vi "Stop Condition - Saturation 4 (SubVI) (1).vi"(6 "Enum":T1(ring), 8 "error in (no error)":errorcluster, 9 "Time":dbl, 11 "Cluster in":T2 {"M Event" items=["Stop", "Running", "PID", "Up Limit", "Down Limit", "Load Limit"]; "Test Type" items=["Please Select", "Triaxial Shear", "Triaxial UU", "Shearbox", "Permeability", "Consolidation (Stepped Loading)/Swelling", "Saturation (Incremental)", "User Defined", "UCT", "Isotropic Consolidation", "Swelling Pressure", "B-Check", "Saturation (Step Increment)", "Saturation (Ramp)"]; "Data"."Test Type" items=["Please Select", "Triaxial Shear", "Triaxial UU", "Shearbox", "Permeability", "Consolidation (Stepped Loading)/Swelling", "Saturation (Incremental)", "User Defined", "UCT", "Isotropic Consolidation", "Swelling Pressure", "B-Check", "Saturation (Step Increment)", "Saturation (Ramp)"]}) -> (0 "error out":errorcluster, 3 "Cluster out":T2 {"M Event" items=["Stop", "Running", "PID", "Up Limit", "Down Limit", "Load Limit"]; "Test Type" items=["Please Select", "Triaxial Shear", "Triaxial UU", "Shearbox", "Permeability", "Consolidation (Stepped Loading)/Swelling", "Saturation (Incremental)", "User Defined", "UCT", "Isotropic Consolidation", "Swelling Pressure", "B-Check", "Saturation (Step Increment)", "Saturation (Ramp)"]; "Data"."Test Type" items=["Please Select", "Triaxial Shear", "Triaxial UU", "Shearbox", "Permeability", "Consolidation (Stepped Loading)/Swelling", "Saturation (Incremental)", "User Defined", "UCT", "Isotropic Consolidation", "Swelling Pressure", "B-Check", "Saturation (Step Increment)", "Saturation (Ramp)"]}, 4 "Delay":string, 7 "Log?":bool)   [LabVIEW 2019]
uses:
  Controls/RunTest - Data Structure.ctl
  Controls/Test Panel - Data Structure.ctl
  Controls/Station - Test Type.ctl
  <vilib>/Utility/miscctls.llb/LVRowAndColumnTypeDef.ctl
  Controls/RunTest - Calculate Data.ctl
  <vilib>/httpClient/ClientHandle.ctl
  Controls/RunTest - Start Condition.ctl
  Controls/RunTest - Stop Condition.ctl
  Controls/UDP - Event.ctl
  Controls/RunTest - State.ctl
  Controls/eFGV States.ctl
  <vilib>/httpClient/LabVIEWHTTPClient.lvlib
types:
  T1 = enum16{"Saturation", "B-Check", "Sat Step", "Sat Ramp"}
  T2 = typedef "RunTest - Data Structure.ctl" = cluster{"Test Plan":string[], "PlanRow":i32, "Device Name":string[], "Timeout":i32, "Start?":bool, "Pause?":bool, "IP Address":string[], "LogRow":i32, "Logtype":u16, "Log Elapse":sgl, "Data":T3, "Stop log?":bool, "tdms":refnum<k34>, "Sensor Data":sgl[], "Start time":timestamp, "Prev Log Elapse":u32, "Plot":u16, "X-Axis":u16[], "Y-Axis":u16[], "XY":cluster{"X":dbl, "Y":dbl}[][], "End Stage?":bool, "1run":bool, "Condition":u16[], "Start Con":bool, "Log Con":bool, "Stop Con":bool, "Start Elapse":dbl, "Start Load":dbl, "Motor":i32, "StartRow":i32, "number log":i32, "Dir":bool, "Start time test":timestamp, "Auto":bool, "Check return?":bool, "Inv":cluster{"M":i32[], "Bool":bool[]}, "tdms temp":refnum<k34>, "Zero?":bool, "Plot Timer":dbl, "1st Run":bool, "TDMS Path":path, "MaxLoad":dbl, "Log Timer":sgl[], "Test Type":T4, "Log Sensor":string[], "Save?":bool, "1st Log":bool, "Y-Axis 2":u16[], "On Y-Axis 2":bool, "Decimal":u8[], "Init":cluster{"PWP TS":sgl, "Load TS":sgl, "Volume TS":sgl, "Disp TS":sgl, "CP":sgl, "Vol In":sgl, "Vol Out":sgl, "Load UCT":sgl, "Disp UCT":sgl, "PWP Sat":sgl, "CP Sat":sgl, "Volume IsoCons":sgl, "PWP IsoCons":sgl, "PWP TUU":sgl, "Load TUU":sgl, "Volume TUU":sgl, "Disp TUU":sgl, "Load Cons":sgl, "Disp Cons":sgl, "Volume Sat":sgl, "Vertical Load SB":sgl, "Vertical Disp SB":sgl, "H Disp SB":sgl, "H Load SB":sgl, "PWP BC":sgl, "CP BC":sgl, "PWP Sat Step":sgl, "CP Sat Step":sgl, "Volume Sat Step":sgl, "PWP Sat Ramp":sgl, "CP Sat Ramp":sgl, "Volume Sat Ramp":sgl}, "Calc":T6, "Device Index":i32[], "Channel Index":i32[], "http ref":T7, "fileid":string, "Step Cons":cluster{"V Stress":sgl, "H Settlement":sgl}, "RunTest":bool, "Graph Last":i32, "Init?":bool, "Datalog":bool[], "Start":T8, "Stop":T9, "Running?":bool, "StartTime":dbl, "Log Prev Time":dbl, "KeyName":string[], "Test RunTime":dbl, "Log Prev Axial":dbl, "M Event":T10[], "Last Log":bool, "popup":bool, "PreStart UU":bool, "PreStart Sat":bool, "PreStart BC":bool, "PreStart Sat Step":bool, "PreStart Sat Ramp":bool, "Prev Sat IP":string}
  T3 = typedef "Test Panel - Data Structure.ctl" = cluster{"Station":string, "Sample ID":string, "Job No":string, "Job Description":string, "Filename":string, "Test Type":T4, "Speciment No":string, "Depth":string, "Height":string, "Diameter/Length":string, "Weight":string, "Test Parameter":string, "Station[]":string[], "Edit Pos":T5, "Edit Pos Prev":T5, "Area":string, "Path":string, "sample_id":string}
  T4 = typedef "Station - Test Type.ctl" = u16
  T5 = typedef "LVRowAndColumnTypeDef.ctl" = cluster{"Row":i32, "Column":i32}
  T6 = typedef "RunTest - Calculate Data.ctl" = cluster{"TS":cluster{"Change PWP":sgl, "Change Vol":sgl, "Axial Load":sgl, "CiL":sgl, "Deviator":sgl, "Axial Strain":sgl, "MaxDeviator":sgl, "SS":sgl, "CAS":sgl}, "TUU":cluster{"Change PWP":sgl, "Axial Load":sgl, "CiL":sgl, "Deviator":sgl, "Axial Strain":sgl, "MaxDeviator":sgl}, "Sat":cluster{"B Value":sgl, "PWP Diss":sgl, "CPP":sgl, "CV":sgl}, "Per":cluster{"Change Vol In":sgl, "Change Vol Out":sgl, "Mean Vol":sgl, "Gradient Pressure":sgl, "Outlet Flow":sgl, "Inlet Flow":sgl, "I X1":sgl, "I X2":sgl, "I Y1":sgl, "I Y2":sgl, "O X1":sgl, "O X2":sgl, "O Y1":sgl, "O Y2":sgl}, "Step Cons":cluster{"V Stress":sgl, "H Settlement":sgl, "Total H Settle":sgl, "Prev Total H":sgl}, "UCT":cluster{"ALC":sgl, "H Change":sgl, "Deviator":sgl, "Axial Strain":sgl, "V Stress":sgl, "MaxDeviator":sgl}, "ISO Cons":cluster{"CPP":sgl, "PWP Diss":sgl, "CV":sgl, "VS":sgl}, "SB":cluster{"Speci LenC":sgl, "Shear Strain":sgl, "H LC":sgl, "Normal Stress":sgl, "Shear Stress":sgl, "MaxShear":sgl}, "BC":cluster{"B Value":sgl, "PWP Diss":sgl, "CPP":sgl, "CV":sgl}, "Sat Step":cluster{"B Value":sgl, "PWP Diss":sgl, "CPP":sgl, "CV":sgl}, "Sat Ramp":cluster{"B Value":sgl, "PWP Diss":sgl, "CPP":sgl, "CV":sgl}, "Prev Log":string[]}
  T7 = typedef "LabVIEWHTTPClient.lvlib/ClientHandle.ctl" = refnum<k1>
  T8 = typedef "RunTest - Start Condition.ctl" = cluster{"Cons":cluster{"VS":dbl, "Delay":bool, "No Delay":dbl}, "Sat":cluster{"CP":dbl, "BP":dbl, "StartBP":bool, "Target CP":bool, "Target BP":bool}, "Iso":cluster{"Select":dbl, "BP":dbl, "IC2":dbl, "IC3":dbl, "IC4":dbl, ". IC6":bool, "IC6":dbl, "IC6-2":dbl, "Time Cond":dbl, "Last PWP":dbl, "Target CP":bool, "Target BP":bool, "NewCP":dbl, "NewBP":dbl, "Noti CP":bool, "Noti BP":bool, "Noti PWP":bool, "PrevSatBP":dbl}, "TS":cluster{"SS":dbl, "Engage":bool, "ES":dbl, "LC":dbl, "PreStart":bool, "Trig SS":bool, "Drain":dbl, "Select":u16, "Max SS .":bool, "MaxSS":dbl}, "TUU":cluster{"SS":dbl, "Engage":bool, "ES":dbl, "LC":dbl, "PreStart":bool, "Trig SS":bool, "CP":dbl, "Delay Value":dbl, "Delay":bool, "CP PID":bool}, "UCT":cluster{"SS":dbl, "Engage":bool, "ES":dbl, "LC":dbl, "PreStart":bool, "Trig SS":bool}, "Enable?":bool, "SB":cluster{"SS":dbl, "Engage":bool, "ES":dbl, "LC":dbl, "PreStart":bool, "Trig SS":bool, "VS":dbl, "Delay Value":dbl, "Delay":bool, "VS PID":bool}, "Perm":cluster{"DP":dbl}, "BC":cluster{"CP":dbl, "Target CP":bool, "Target BP":bool, "CP Inc":dbl, "CP .Init":bool, "CP Init":dbl, "1st BC":bool}, "Sat (Step)":cluster{"Select":dbl, "CP":dbl, "BP":dbl, "EP":dbl, "StartCP":bool, "Target CP":bool, "Target BP":bool}, "Sat (Ramp)":cluster{"Select":dbl, "CP":dbl, "BP":dbl, "EP":dbl, "StartCP":bool, "Target CP":bool, "Target BP":bool, "Time Rate":u32}}
  T9 = typedef "RunTest - Stop Condition.ctl" = cluster{"Cons":cluster{"Select":i32, "Disp":dbl, "Time":dbl, "Time2":dbl, "Disp 2":dbl, "Time Cond":dbl, "Last Disp":dbl, "Swell":bool, "T50,90,100":cluster{"t50_x_min":dbl, "t50_y_value":dbl, "t90_x_min":dbl, "t90_y_value":dbl, "t100_x_min":dbl, "t100_y_value":dbl, "target_column":string, "test_type":string, "error":string}}, "Sat":cluster{"Select":i32, "PP":dbl, "Time":dbl, "VC":dbl, "Time2":dbl, "Time Cond":dbl, "Last PP":dbl, ".B":bool, "B":dbl, "Last Vc":dbl, "Time Cond 2":dbl, "Time3":dbl, "Time Cond 3":dbl, "B Achieve":bool, "PP Achieve":bool, "VC Achieve":bool, "Max Achieve":bool, "CP Check":dbl, "Skip Next":bool, "B Achieve Stage":u32, ".CP Check":bool}, "Iso":cluster{"PP":dbl, "Time":dbl, "VC":dbl, "Time2":dbl, "Time Cond":dbl, "Last Vc":dbl, ".PP":bool, "Time Cond 2":dbl, "Select":i32, "BS":cluster{"t50_x_min":dbl, "t50_y_value":dbl, "t90_x_min":dbl, "t90_y_value":dbl, "t100_x_min":dbl, "t100_y_value":dbl, "target_column":string, "test_type":string, "error":string}, "Final VC":dbl, "ASTM":cluster{"t50_x_min":dbl, "t50_y_value":dbl, "t90_x_min":dbl, "t90_y_value":dbl, "t100_x_min":dbl, "t100_y_value":dbl, "target_column":string, "test_type":string, "error":string}, "ASTM Log":cluster{"t50_x_min":dbl, "t50_y_value":dbl, "t90_x_min":dbl, "t90_y_value":dbl, "t100_x_min":dbl, "t100_y_value":dbl, "target_column":string, "test_type":string, "error":string}, "PP Achieve":bool, "VC Achieve":bool}, "TS":cluster{"Axial":dbl, ".MaxDev":bool, "MaxDev Value":dbl, "Return":bool, "Reset":bool, "Prev Time":dbl, "PostStop Run":bool, "CP Stop":bool, "BP Stop":bool, "PostStop Trig":bool, "Reset Value":dbl, "BPTrig":bool, "CPTrig":bool, "VLCTrig":bool, "CAxial":dbl, "Select":i32}, "TUU":cluster{"Axial":dbl, ".MaxDev":bool, "MaxDev Value":dbl, "Return":bool, "Reset":bool, "Prev Time":dbl, "PostStop Run":bool, "CP Stop":bool, "BP Stop":bool, "PostStop Trig":bool, "Reset Value":dbl, "BPTrig":bool, "CPTrig":bool, "VLCTrig":bool}, "UCT":cluster{"Axial":dbl, ".MaxDev":bool, "MaxDev Value":dbl, "Return":bool, "Reset":bool, "Prev Time":dbl, "PostStop Run":bool, "CP Stop":bool, "BP Stop":bool, "PostStop Trig":bool}, "Enable?":bool, "SB":cluster{"Shear":dbl, ".MaxShear":bool, "MaxShear Value":dbl, "Return":bool, "Reset":bool, "Prev Time":dbl, "PostStop Run":bool, "CP Stop":bool, "BP Stop":bool, "PostStop Trig":bool, "Reset Value":dbl, "BPTrig":bool, "CPTrig":bool, "VLCTrig":bool}, "Perm":cluster{"Max Time":bool, "Reset":bool, "PostStop Run":bool, "Ratio":bool, "Reset Value":dbl, "Time":dbl, "RatioTime":dbl, "RatioMore":dbl, "RatioLess":dbl, "Time Cond":dbl, "Time Cond 2":dbl, "Prev IF":dbl, "Prev OF":dbl, "PostStop Trig":bool, "BP Trig":bool, "DP Stop":bool, "BP Stop":bool, "CP Stop":bool, "CP Trig":bool}, "SP":cluster{".Max Time":bool, ".Time":bool, "Time":dbl, "MaxTime":dbl, "Time Cond":dbl, "Max Time Cond":dbl, "Stress":dbl}, "BC":cluster{"Select":i32, "PP":dbl, "Time":dbl, "Time Cond":dbl, "Last PP":dbl, ".B":bool, "B":dbl, "Time 2":dbl, "Time Cond 2":dbl, "B Achieve":bool, "PP Achieve":bool, "Max Achieve":bool, "CP Check":dbl, "Skip Next":bool, "B Achieve Stage":u32, ".CP Check":bool}, "Sat (Step)":cluster{"Select":i32, "PP":dbl, "Time":dbl, "VC":dbl, "Time2":dbl, "Time Cond":dbl, "Last PP":dbl, ".B":bool, "B":dbl, "Last Vc":dbl, "Time Cond 2":dbl, "Time3":dbl, "Time Cond 3":dbl, "B Achieve":bool, "PP Achieve":bool, "VC Achieve":bool, "Max Achieve":bool, "CP Check":dbl, "Skip Next":bool, "B Achieve Stage":u32}, "Sat (Ramp)":cluster{"Select":i32, "PP":dbl, "Time":dbl, "VC":dbl, "Time2":dbl, "Time Cond":dbl, "Last PP":dbl, ".B":bool, "B":dbl, "Last Vc":dbl, "Time Cond 2":dbl, "Time3":dbl, "Time Cond 3":dbl, "B Achieve":bool, "PP Achieve":bool, "VC Achieve":bool, "Max Achieve":bool, "CP Check":dbl, "Skip Next":bool, "B Achieve Stage":u32}}
  T10 = typedef "UDP - Event.ctl" = u16
  T11 = typedef "RunTest - State.ctl" = enum16{"Load Testfile", "Notifier", "Init", "Idle", "Load", "Read DB", "Run", "Pause", "Stop", "Check Start", "Check Stop", "Check Post Stop", "Check Log", "EndStage", "Data View", "Data View PWP", "Display", "Graph", "Graph PWP", "Close", "Stop PID", "Check Limit", "Auto", "Up", "Log", "Zero", "Machine Control", "Save Report"}
  T12 = typedef "eFGV States.ctl" = enum16{"Init", "Read", "Write", "Exit"}
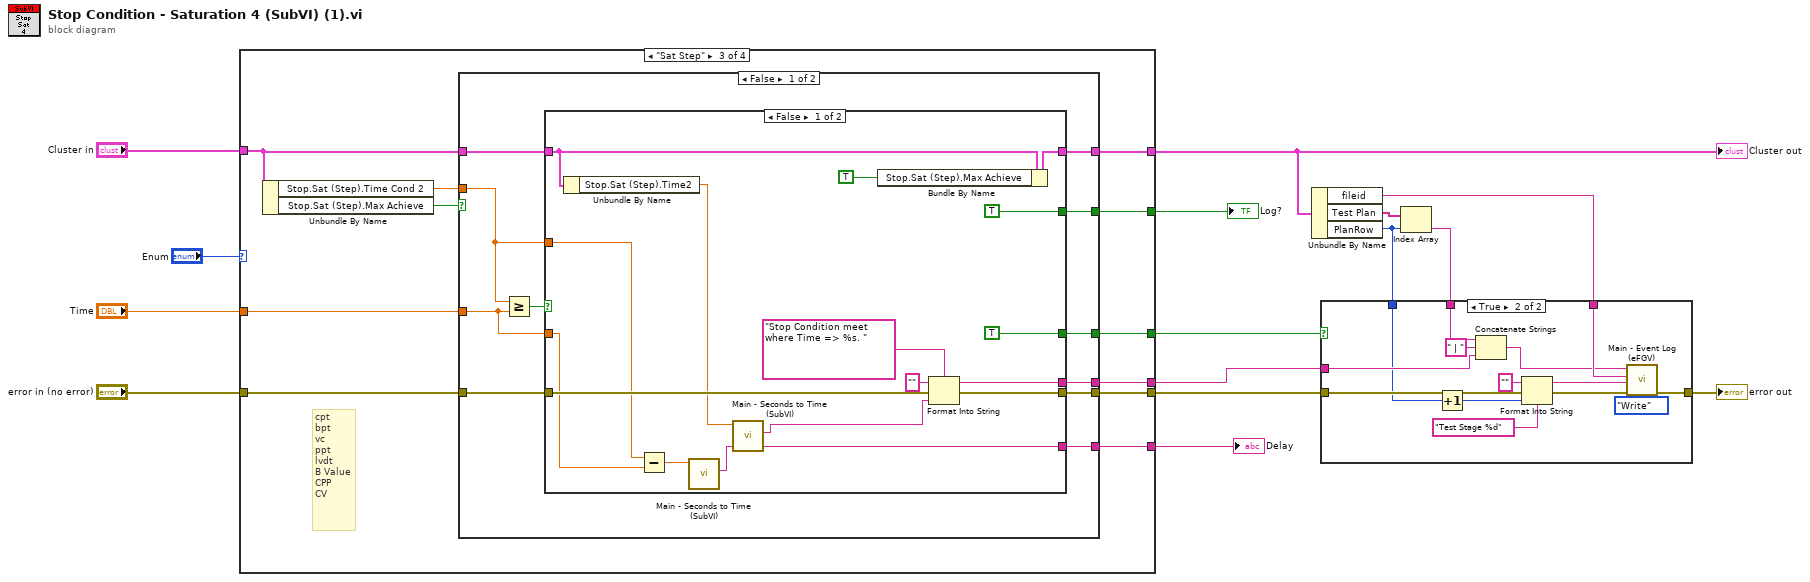
[diagram p0: block diagram]
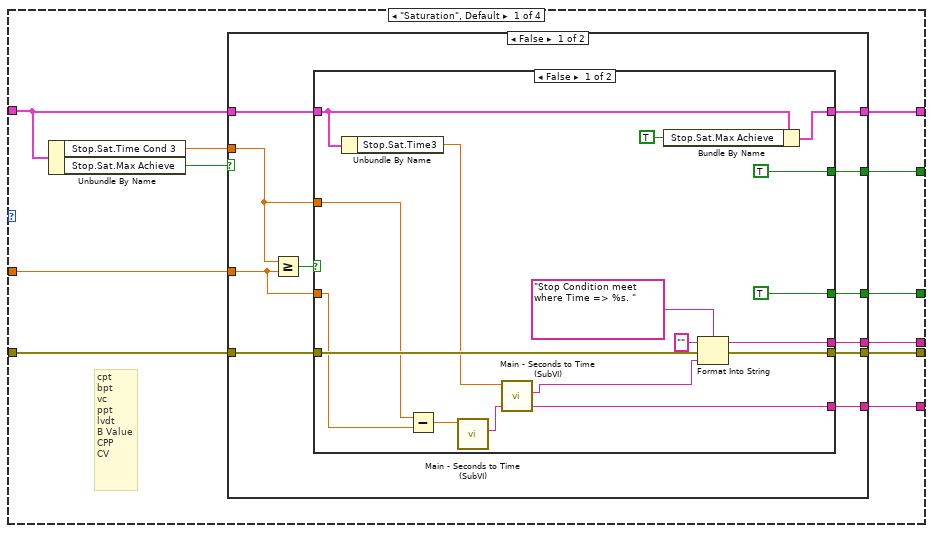
[diagram p2: hidden frame]
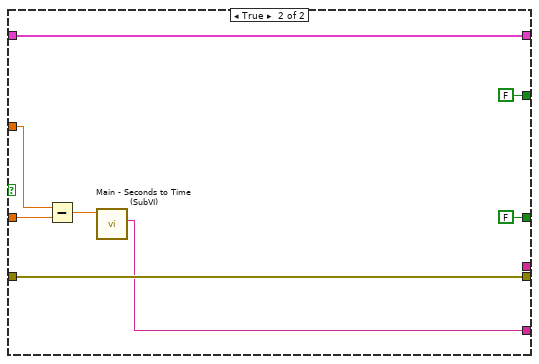
[diagram p3: hidden frame]
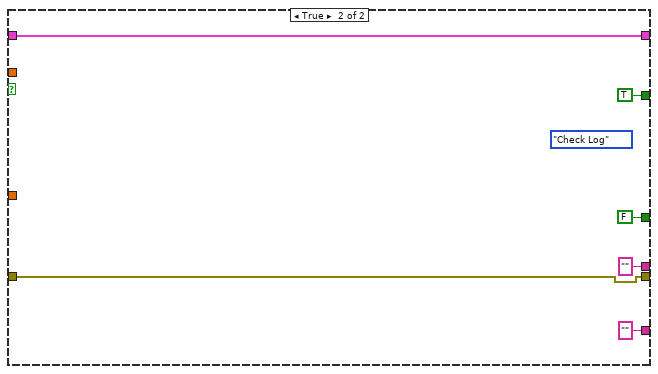
[diagram p4: hidden frame]
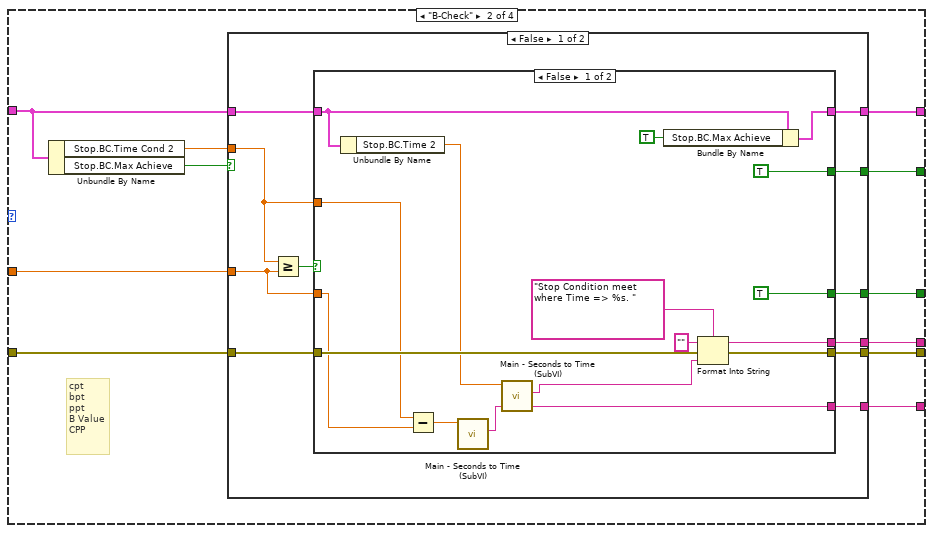
[diagram p5: hidden frame]
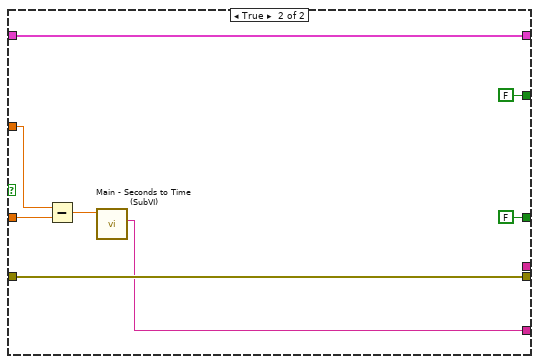
[diagram p6: hidden frame]
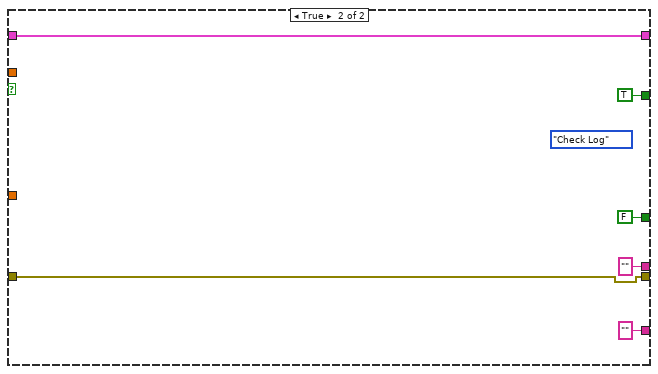
[diagram p7: hidden frame]
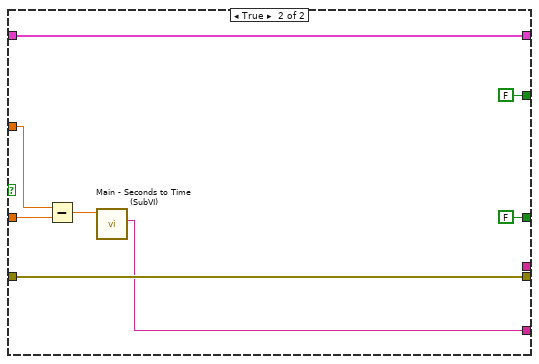
[diagram p8: hidden frame]
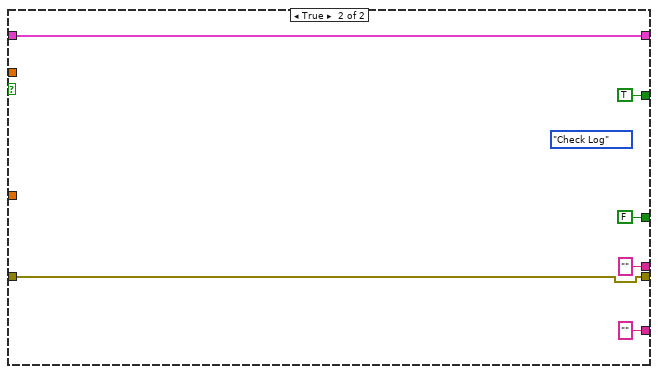
[diagram p9: hidden frame]
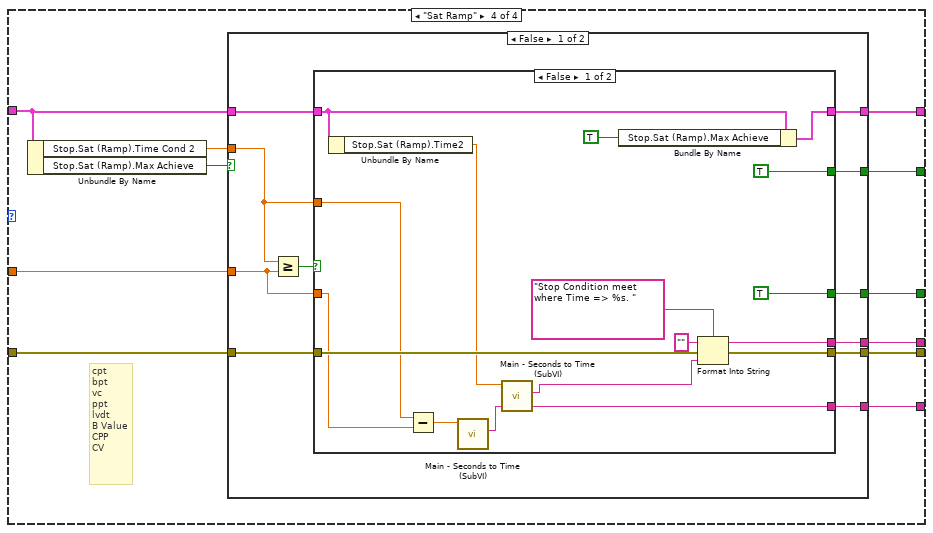
[diagram p10: hidden frame]
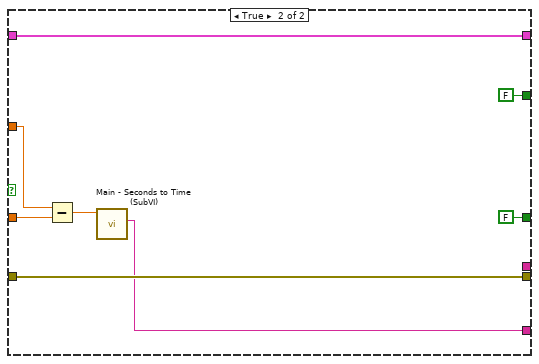
[diagram p11: hidden frame]
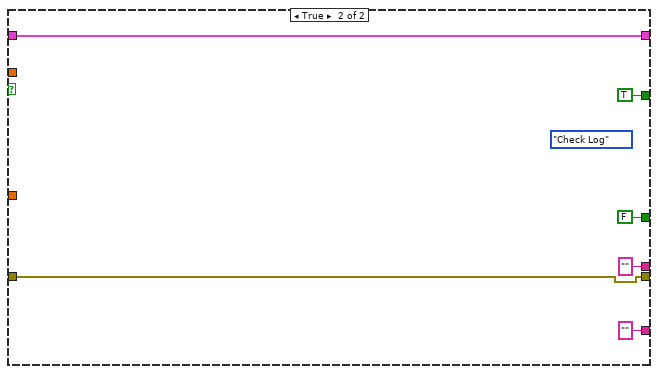
[diagram p12: hidden frame]
diagram:
  n1 = case shown="\"Sat Step\"" "Enum" {
    tunnel: [w26 w78 w130 w182] -> w15
    tunnel: "Time" -> [w25 w77 w129 w181]
    tunnel: "error in (no error)" -> [w24 w76 w128 w180]
    tunnel: "Cluster in" -> [w23 w75 w127 w179]
    tunnel: [w21 w73 w125 w177] -> w11
    tunnel: [w19 w71 w123 w175] -> w6
    tunnel: [w18 w70 w122 w174] -> w5
    tunnel: [w17 w69 w121 w173] -> w4
    tunnel: [w16 w68 w120 w172] -> w3
    frame "Saturation", Default {
      # "cpt\nbpt\nvc\nppt\nlvdt\nB Value\nCPP\nCV"
      n2 = Unbundle By Name(w23) -> ("Stop.Sat.Time Cond 3"=w22:dbl, "Stop.Sat.Max Achieve"=w20:bool)
      n3 = case shown="False" w20 {
        tunnel: [w37 "" ("Time string")] -> w26
        tunnel: w25 -> [w36 _]
        tunnel: [w35 FALSE] -> w18
        tunnel: [w34 ""] -> w16
        tunnel: w24 -> [w33 w63]
        tunnel: [w31 w67] -> w17
        tunnel: [w30 w63] -> w19
        tunnel: w23 -> [w29 w67]
        tunnel: w22 -> [w28 _]
        tunnel: [w27 TRUE] -> w21
        frame False {
          n4 = Greater Or Equal?(x=w28, y=w36) -> (x >= y?=w32:bool)
          n5 = case shown="False" w32 {
            tunnel: [w51 w61] -> w30
            tunnel: w33 -> [w52 w61]
            tunnel: [w40 w60] -> w31
            tunnel: w29 -> [w39 w60]
            tunnel: w28 -> [w45 w57]
            tunnel: [w50 _] -> w34
            tunnel: [TRUE FALSE] -> w35
            tunnel: w36 -> [w44 w56]
            tunnel: [w43 w55] -> w37
            tunnel: [TRUE FALSE] -> w27
            frame False {
              n6 = Unbundle By Name(w39) -> ("Stop.Sat.Time3"=w42:dbl)
              n7 = Subtract(x=w45, y=w44) -> (x-y=w46:dbl)
              n8 = call "Main - Seconds to Time (SubVI).vi"("Seconds"=w46) -> ("Time string"=w43:string)  [unwired: 9 in, 1 out]
              n9 = call "Main - Seconds to Time (SubVI).vi"("Seconds"=w42) -> ("Time string"=w47:string)  [unwired: 9 in, 1 out]
              n10 = Bundle By Name(cluster=w39, "Stop.Sat.Max Achieve"=TRUE) -> (w40:T2)
              n11 = Format Into String(format string="Stop Condition meet where Time => %s. ", initial string="", error in=w52, w47) -> (resulting string=w50:string, error out=w51:errorcluster)
            }
            frame True {
              n12 = Subtract(x=w57, y=w56) -> (x-y=w58:dbl)
              n13 = call "Main - Seconds to Time (SubVI).vi"("Seconds"=w58) -> ("Time string"=w55:string)  [unwired: 9 in, 1 out]
            }
          }
        }
        frame True {
          (unwired) RunTest_-_State."Check Log"
        }
      }
    }
    frame "B-Check" {
      # "cpt\nbpt\nppt\nB Value\nCPP"
      n14 = Unbundle By Name(w75) -> ("Stop.BC.Time Cond 2"=w74:dbl, "Stop.BC.Max Achieve"=w72:bool)
      n15 = case shown="False" w72 {
        tunnel: [w89 "" ("Time string")] -> w78
        tunnel: w77 -> [w88 _]
        tunnel: [w87 FALSE] -> w70
        tunnel: [w86 ""] -> w68
        tunnel: w76 -> [w85 w115]
        tunnel: [w83 w119] -> w69
        tunnel: [w82 w115] -> w71
        tunnel: w75 -> [w81 w119]
        tunnel: w74 -> [w80 _]
        tunnel: [w79 TRUE] -> w73
        frame False {
          n16 = Greater Or Equal?(x=w80, y=w88) -> (x >= y?=w84:bool)
          n17 = case shown="False" w84 {
            tunnel: [w103 w113] -> w82
            tunnel: w85 -> [w104 w113]
            tunnel: [w92 w112] -> w83
            tunnel: w81 -> [w91 w112]
            tunnel: w80 -> [w97 w109]
            tunnel: [w102 _] -> w86
            tunnel: [TRUE FALSE] -> w87
            tunnel: w88 -> [w96 w108]
            tunnel: [w95 w107] -> w89
            tunnel: [TRUE FALSE] -> w79
            frame False {
              n18 = Unbundle By Name(w91) -> ("Stop.BC.Time 2"=w94:dbl)
              n19 = Subtract(x=w97, y=w96) -> (x-y=w98:dbl)
              n20 = call "Main - Seconds to Time (SubVI).vi"("Seconds"=w98) -> ("Time string"=w95:string)  [unwired: 9 in, 1 out]
              n21 = call "Main - Seconds to Time (SubVI).vi"("Seconds"=w94) -> ("Time string"=w99:string)  [unwired: 9 in, 1 out]
              n22 = Bundle By Name(cluster=w91, "Stop.BC.Max Achieve"=TRUE ("Stop.Sat.Max Achieve")) -> (w92:T2)
              n23 = Format Into String(format string="Stop Condition meet where Time => %s. ", initial string="", error in=w104, w99) -> (resulting string=w102:string, error out=w103:errorcluster)
            }
            frame True {
              n24 = Subtract(x=w109, y=w108) -> (x-y=w110:dbl)
              n25 = call "Main - Seconds to Time (SubVI).vi"("Seconds"=w110) -> ("Time string"=w107:string)  [unwired: 9 in, 1 out]
            }
          }
        }
        frame True {
          (unwired) RunTest_-_State."Check Log"
        }
      }
    }
    frame "Sat Step" {
      # "cpt\nbpt\nvc\nppt\nlvdt\nB Value\nCPP\nCV"
      n26 = Unbundle By Name(w127) -> ("Stop.Sat (Step).Time Cond 2"=w126:dbl, "Stop.Sat (Step).Max Achieve"=w124:bool)
      n27 = case shown="False" w124 {
        tunnel: [w141 "" ("Time string")] -> w130
        tunnel: w129 -> [w140 _]
        tunnel: [w139 FALSE] -> w122
        tunnel: [w138 ""] -> w120
        tunnel: w128 -> [w137 w167]
        tunnel: [w135 w171] -> w121
        tunnel: [w134 w167] -> w123
        tunnel: w127 -> [w133 w171]
        tunnel: w126 -> [w132 _]
        tunnel: [w131 TRUE] -> w125
        frame False {
          n28 = Greater Or Equal?(x=w132, y=w140) -> (x >= y?=w136:bool)
          n29 = case shown="False" w136 {
            tunnel: [w155 w165] -> w134
            tunnel: w137 -> [w156 w165]
            tunnel: [w144 w164] -> w135
            tunnel: w133 -> [w143 w164]
            tunnel: w132 -> [w149 w161]
            tunnel: [w154 _] -> w138
            tunnel: [TRUE FALSE] -> w139
            tunnel: w140 -> [w148 w160]
            tunnel: [w147 w159] -> w141
            tunnel: [TRUE FALSE] -> w131
            frame False {
              n30 = Unbundle By Name(w143) -> ("Stop.Sat (Step).Time2"=w146:dbl)
              n31 = Subtract(x=w149, y=w148) -> (x-y=w150:dbl)
              n32 = call "Main - Seconds to Time (SubVI).vi"("Seconds"=w150) -> ("Time string"=w147:string)  [unwired: 9 in, 1 out]
              n33 = call "Main - Seconds to Time (SubVI).vi"("Seconds"=w146) -> ("Time string"=w151:string)  [unwired: 9 in, 1 out]
              n34 = Bundle By Name(cluster=w143, "Stop.Sat (Step).Max Achieve"=TRUE ("Stop.Sat.Max Achieve")) -> (w144:T2)
              n35 = Format Into String(format string="Stop Condition meet where Time => %s. ", initial string="", error in=w156, w151) -> (resulting string=w154:string, error out=w155:errorcluster)
            }
            frame True {
              n36 = Subtract(x=w161, y=w160) -> (x-y=w162:dbl)
              n37 = call "Main - Seconds to Time (SubVI).vi"("Seconds"=w162) -> ("Time string"=w159:string)  [unwired: 9 in, 1 out]
            }
          }
        }
        frame True {
          (unwired) RunTest_-_State."Check Log"
        }
      }
    }
    frame "Sat Ramp" {
      # "cpt\nbpt\nvc\nppt\nlvdt\nB Value\nCPP\nCV"
      n38 = Unbundle By Name(w179) -> ("Stop.Sat (Ramp).Time Cond 2"=w178:dbl, "Stop.Sat (Ramp).Max Achieve"=w176:bool)
      n39 = case shown="False" w176 {
        tunnel: [w193 "" ("Time string")] -> w182
        tunnel: w181 -> [w192 _]
        tunnel: [w191 FALSE] -> w174
        tunnel: [w190 ""] -> w172
        tunnel: w180 -> [w189 w219]
        tunnel: [w187 w223] -> w173
        tunnel: [w186 w219] -> w175
        tunnel: w179 -> [w185 w223]
        tunnel: w178 -> [w184 _]
        tunnel: [w183 TRUE] -> w177
        frame False {
          n40 = Greater Or Equal?(x=w184, y=w192) -> (x >= y?=w188:bool)
          n41 = case shown="False" w188 {
            tunnel: [w207 w217] -> w186
            tunnel: w189 -> [w208 w217]
            tunnel: [w196 w216] -> w187
            tunnel: w185 -> [w195 w216]
            tunnel: w184 -> [w201 w213]
            tunnel: [w206 _] -> w190
            tunnel: [TRUE FALSE] -> w191
            tunnel: w192 -> [w200 w212]
            tunnel: [w199 w211] -> w193
            tunnel: [TRUE FALSE] -> w183
            frame False {
              n42 = Unbundle By Name(w195) -> ("Stop.Sat (Ramp).Time2"=w198:dbl)
              n43 = Subtract(x=w201, y=w200) -> (x-y=w202:dbl)
              n44 = call "Main - Seconds to Time (SubVI).vi"("Seconds"=w202) -> ("Time string"=w199:string)  [unwired: 9 in, 1 out]
              n45 = call "Main - Seconds to Time (SubVI).vi"("Seconds"=w198) -> ("Time string"=w203:string)  [unwired: 9 in, 1 out]
              n46 = Bundle By Name(cluster=w195, "Stop.Sat (Ramp).Max Achieve"=TRUE ("Stop.Sat.Max Achieve")) -> (w196:T2)
              n47 = Format Into String(format string="Stop Condition meet where Time => %s. ", initial string="", error in=w208, w203) -> (resulting string=w206:string, error out=w207:errorcluster)
            }
            frame True {
              n48 = Subtract(x=w213, y=w212) -> (x-y=w214:dbl)
              n49 = call "Main - Seconds to Time (SubVI).vi"("Seconds"=w214) -> ("Time string"=w211:string)  [unwired: 9 in, 1 out]
            }
          }
        }
        frame True {
          (unwired) RunTest_-_State."Check Log"
        }
      }
    }
  }
  "Delay" <- w15
  "Cluster out" <- w4
  "Log?" <- w11
  n50 = Unbundle By Name(w4) -> ("fileid"=w8:string, "Test Plan"=w9:string[], "PlanRow"=w7:i32)
  n51 = Index Array(array=w9, index=w7) -> (element=w10:string)
  n52 = case shown="True" w5 {
    tunnel: w6 -> [w224 w228]
    tunnel: [w224 w237] -> w2
    tunnel: w8 -> [_ w236]
    tunnel: w3 -> [_ w232]
    tunnel: w10 -> [_ w235]
    tunnel: w7 -> [_ w226]
    frame False {
    }
    frame True {
      n53 = Increment(x=w226) -> (x+1=w230:i32)
      n54 = Concatenate Strings(w235, " | " ("string"), w232) -> (w233:string)
      n55 = Format Into String(format string="Test Stage %d", initial string="", error in=w228, w230) -> (resulting string=w227:string, error out=w229:errorcluster)
      n56 = call "Main - Event Log (eFGV).vi"("Action"=eFGV_States."Write", "error in"=w229, "Stage"=w227, "Fileid"=w236, "Data In"=w233) -> ("error out"=w237:errorcluster)  [unwired: 3 in, 3 out]
    }
  }
  "error out" <- w2
